vi "Leave Process Loop.vi"(8 "error in (no error)":errorcluster, 11 "Process In":refnum<class "Process.lvclass">) -> (0 "error out":errorcluster, 3 "Process Out":refnum<class "Process.lvclass">)   [LabVIEW 2020, in "Process.lvclass"]
doc: "Forces clearing of the in process loop flag, which is carried by value. This VI should be called if a branch of the process instance is sent out of the process loop to gurantee that the Get Lifecycle State.vi returns the correct result."
uses:
  Process.lvclass
  Process.lvclass/Process.ctl
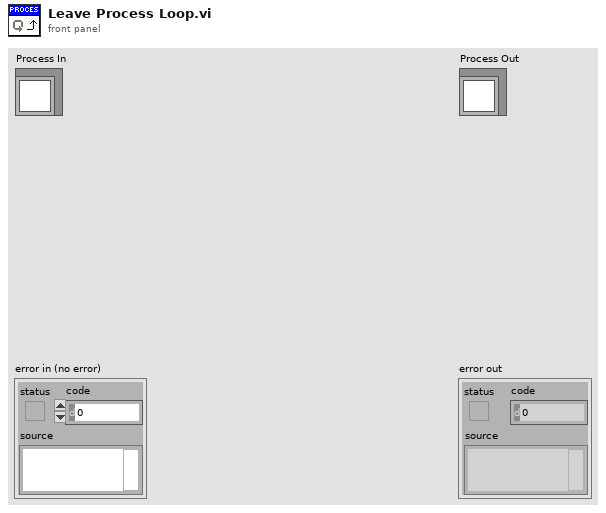
[diagram p1: front panel]
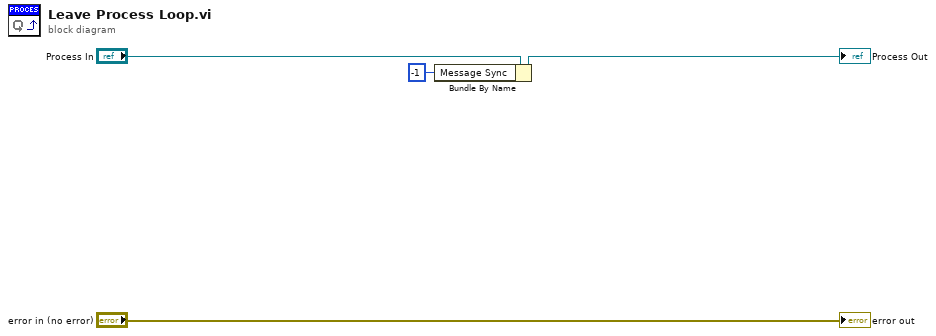
[diagram p0: block diagram]
diagram:
  n1 = Bundle By Name(cluster="Process In", "Message Sync"=-1) -> (→"Process Out":refnum<class "Process.lvclass">)
  "error out" <- "error in (no error)"
